vi "Render Template.vi"(6 "Locals (None)":refnum<class "Value Tree.lvclass">, 7 "Folder":path, 8 "error in (no error)":errorcluster, 10 "Template":string, 11 "BasicTemplater in":refnum<class "BasicTemplater.lvclass">) -> (0 "error out":errorcluster, 2 "Output":string, 3 "BasicTemplater out":refnum<class "BasicTemplater.lvclass">)   [LabVIEW 2020, in "HTTP Server.lvlib" / "BasicTemplater.lvclass"]
uses:
  BasicTemplater.lvclass
  Value Tree/Value Tree.lvclass
  Value Tree/Value Tree.lvclass/Value Tree.ctl
  BasicTemplater.lvclass/BasicTemplater.ctl
  Value Tree/Create.vi
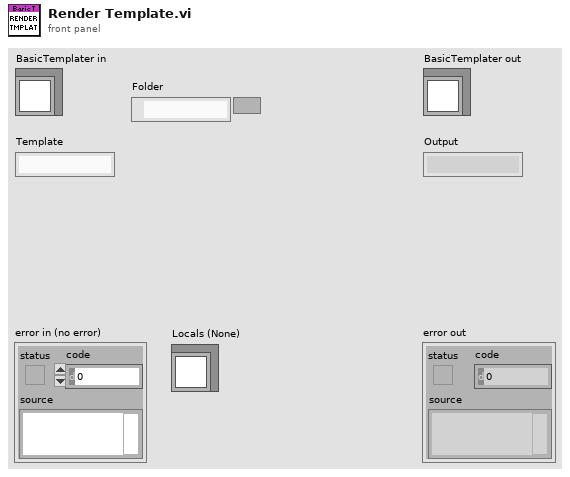
[diagram p1: front panel]
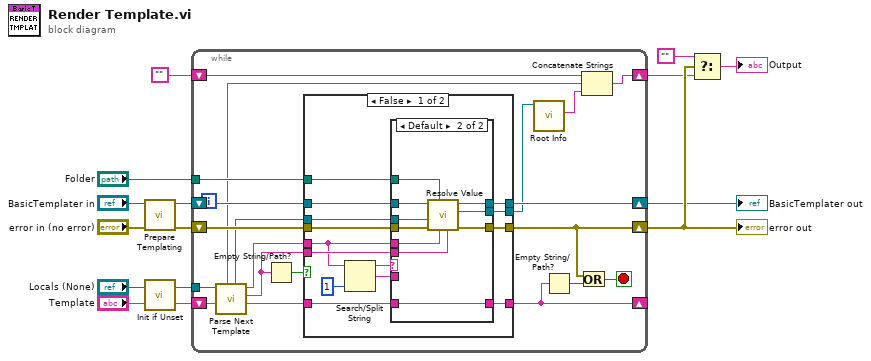
[diagram p0: block diagram]
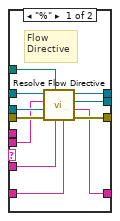
[diagram p2: hidden frame]
diagram:
  n1 = call "Prepare Templating.vi"("error in (no error)"="error in (no error)", "BasicTemplater in"="BasicTemplater in") -> ("error out"=w8:errorcluster, "BasicTemplater out"=w10:refnum<class "BasicTemplater.lvclass">)  [unwired: 8 in]
  n2 = call "Init if Unset.vi"("Value Tree in"="Locals (None)") -> ("Value Tree out"=w1:refnum<class "Value Tree.lvclass">)  [unwired: 6 in]
  n3 = while {
    shift-right: [w32] -> w7
    shift-left: "" -> [w33]
    shift-right: [w15] -> _
    shift-left: "Template" -> [w29]
    shift-right: [w30] -> w11
    shift-left: w10 -> [w31]
    shift-right: [w26] -> w14
    shift-left: w8 -> [w34]
    tunnel: "Folder" -> [w24]
    tunnel: w1 -> [w19]
    stop <- w27 stop-if-true
    n4 = call "Parse Next Template.vi"("Text"=w29, "Locals in"=w19) -> ("Remaining"=w16:string, "Value Name"=w21:string, "Namespace"=w22:string, "Locals"=w20:refnum<class "Value Tree.lvclass">, "Before"=w23:string)  [unwired: 5 in]
    n5 = Empty String/Path?(string/path=w21) -> (empty?=w25:bool)
    n6 = case shown="False" w25 {
      tunnel: w34 -> [w48 w71]
      tunnel: w31 -> [w47 w72]
      tunnel: [w46 _] -> w18
      tunnel: [w45 w72] -> w30
      tunnel: [w44 w71] -> w26
      tunnel: w24 -> [w43 _]
      tunnel: w22 -> [w39 _]
      tunnel: w21 -> [w42 _]
      tunnel: w20 -> [w41 _]
      tunnel: w16 -> [w37 w70]
      tunnel: [w35 w70] -> w15
      frame False {
        n7 = Search/Split String(string=w39, offset (0)=1) -> (substring before match=w38:string, match + rest of string=w36:string)  [unwired: 1 in, 1 out]
        n8 = case shown="Default" w38 {
          tunnel: w48 -> [w57 w69]
          tunnel: w47 -> [w59 w68]
          tunnel: [w54 w67] -> w46
          tunnel: [w55 w66] -> w45
          tunnel: [w53 w65] -> w44
          tunnel: w43 -> [w56 w64]
          tunnel: w42 -> [w49 w63]
          tunnel: w41 -> [w58 w62]
          tunnel: w39 -> [_ w61]
          tunnel: w37 -> [w52 w60]
          tunnel: w36 -> [w50 _]
          tunnel: [w51 w60] -> w35
          frame "%" {
            # "Flow Directive"
            n9 = call "Resolve Flow Directive.vi"("Remaining in"=w52, "Directive"=w50, "Folder"=w56, "error in (no error)"=w57, "Locals in"=w58, "Value Name"=w49, "BasicTemplater in"=w59) -> ("error out"=w53:errorcluster, "Remaining"=w51:string, "Value"=w54:refnum<class "Value Tree.lvclass">, "BasicTemplater out"=w55:refnum<class "BasicTemplater.lvclass">)  [unwired: 1 in]
          }
          frame Default {
            n10 = call "Resolve Value.vi"("Value Name"=w63, "Namespace"=w61, "Folder"=w64, "error in (no error)"=w69, "Locals in"=w62, "BasicTemplater in"=w68) -> ("error out"=w65:errorcluster, "Value"=w67:refnum<class "Value Tree.lvclass">, "BasicTemplater out"=w66:refnum<class "BasicTemplater.lvclass">)  [unwired: 3 in]
          }
        }
      }
      frame True {
      }
    }
    n11 = call "Root Info.vi"("Value Tree in"=w18) -> ("Value"=w17:string)  [unwired: 6 in, 4 out]
    n12 = Empty String/Path?(string/path=w15) -> (empty?=w28:bool)
    n13 = Or(x=w26, y=w28) -> (x .or. y?=w27:bool)
    n14 = Concatenate Strings(w33, w23, w17) -> (w32:string)
  }
  "error out" <- w14
  "BasicTemplater out" <- w11
  n15 = Select(t="", s=w14, f=w7) -> (s? t:f=→"Output":string)
